vi "CANsub_Check_Version.vi"(8 "error in (no error)":errorcluster, 11 "response":string) -> (0 "error out":errorcluster, 3 "api version":string)   [LabVIEW 2021, in "CANsub_Common.lvlib"]
doc: "Checks that the CANsub API version response is the supported version 05.00 (the constant in this VI). Error 5001: other API version (update the firmware or the client)."
uses:
  CANsub_Common.lvlib
panel:
  out "ok":bool
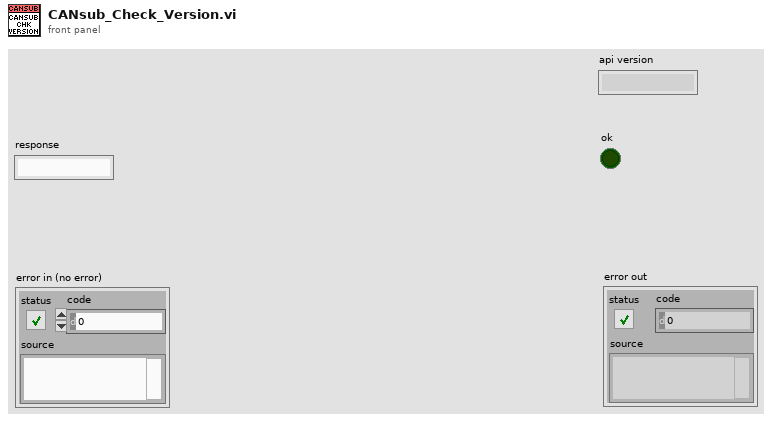
[diagram p1: front panel]
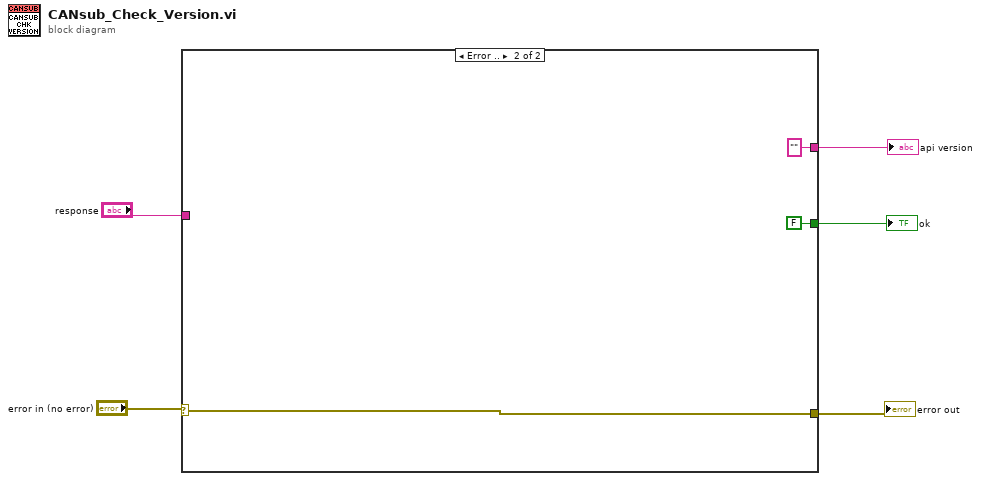
[diagram p0: block diagram]
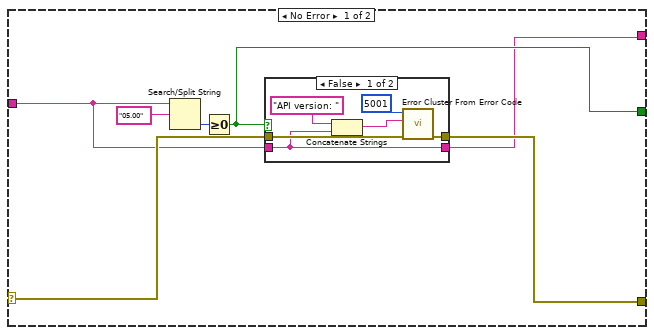
[diagram p2: hidden frame]
diagram:
  n1 = case shown="Error .." "error in (no error)" {
    selector: "error in (no error)" -> [w10 w23]
    tunnel: [w9 w23] -> w5
    tunnel: "response" -> [w8 _]
    tunnel: [w6 "" ("response")] -> w2
    tunnel: [w7 FALSE] -> w1
    frame No Error {
      n2 = Search/Split String(string=w8, search string/char (-)="05.00") -> (offset of match=w12:i32)  [unwired: 1 in, 2 out]
      n3 = Greater Or Equal To 0?(x=w12) -> (x >= 0?=w7:bool)
      n4 = case shown="False" w7 {
        tunnel: w8 -> [w13 w20]
        tunnel: [w13 w20] -> w6
        tunnel: [w15 w19] -> w9
        tunnel: w10 -> [w14 w19]
        frame False {
          n5 = Concatenate Strings("API version: " ("string"), w13) -> (w16:string)
          n6 = call <vilib>:"Error Cluster From Error Code.vi"("error in (no error)"=w14, "error message (\"\")"=w16, "error code (0)"=5001) -> ("error out"=w15:errorcluster)  [unwired: 6 in]
        }
        frame True {
        }
      }
    }
    frame Error {
    }
  }
  "error out" <- w5
  "api version" <- w2
  "ok" <- w1
